vi "eDyno Fault Sequencer.vi"(0 "Automated Sequence":T5={"Run Auto Sequence"=FALSE, "Steps"=[{"Fault Injection"={"Imbalance ON"=FALSE, "Imbalance (g)"=0.5, "Misalignment ON"=FALSE, "Misalignment (g)"=0.2, "Bearing BPFO ON"=FALSE, "Bearing Impact (g)"=2.0, "Motor Ripple ON"=FALSE, "Torque Ripple (g)"=0.3, "PWM Noise ON"=FALSE, "PWM Level (g)"=0.05}, "Speed Profile"={"Run-up Enabled"=TRUE, "Constant Speed (rpm)"=3000.0, "Run-up Start (rpm)"=500.0, "Run-up End (rpm)"=4500.0, "Run-up Duration (s)"=30.0}, "Dwell (s)"=32.0}, {"Fault Injection"={"Imbalance ON"=TRUE, "Imbalance (g)"=0.5, "Misalignment ON"=FALSE, "Misalignment (g)"=0.2, "Bearing BPFO ON"=FALSE, "Bearing Impact (g)"=2.0, "Motor Ripple ON"=FALSE, "Torque Ripple (g)"=0.3, "PWM Noise ON"=FALSE, "PWM Level (g)"=0.05}, "Speed Profile"={"Run-up Enabled"=TRUE, "Constant Speed (rpm)"=3000.0, "Run-up Start (rpm)"=500.0, "Run-up End (rpm)"=4500.0, "Run-up Duration (s)"=30.0}, "Dwell (s)"=32.0}, {"Fault Injection"={"Imbalance ON"=FALSE, "Imbalance (g)"=0.5, "Misalignment ON"=TRUE, "Misalignment (g)"=0.2, "Bearing BPFO ON"=FALSE, "Bearing Impact (g)"=2.0, "Motor Ripple ON"=FALSE, "Torque Ripple (g)"=0.3, "PWM Noise ON"=FALSE, "PWM Level (g)"=0.05}, "Speed Profile"={"Run-up Enabled"=TRUE, "Constant Speed (rpm)"=3000.0, "Run-up Start (rpm)"=500.0, "Run-up End (rpm)"=4500.0, "Run-up Duration (s)"=30.0}, "Dwell (s)"=32.0}, {"Fault Injection"={"Imbalance ON"=FALSE, "Imbalance (g)"=0.5, "Misalignment ON"=FALSE, "Misalignment (g)"=0.2, "Bearing BPFO ON"=TRUE, "Bearing Impact (g)"=2.0, "Motor Ripple ON"=FALSE, "Torque Ripple (g)"=0.3, "PWM Noise ON"=FALSE, "PWM Level (g)"=0.05}, "Speed Profile"={"Run-up Enabled"=TRUE, "Constant Speed (rpm)"=3000.0, "Run-up Start (rpm)"=500.0, "Run-up End (rpm)"=4500.0, "Run-up Duration (s)"=30.0}, "Dwell (s)"=32.0}, {"Fault Injection"={"Imbalance ON"=FALSE, "Imbalance (g)"=0.5, "Misalignment ON"=FALSE, "Misalignment (g)"=0.2, "Bearing BPFO ON"=FALSE, "Bearing Impact (g)"=2.0, "Motor Ripple ON"=TRUE, "Torque Ripple (g)"=0.3, "PWM Noise ON"=FALSE, "PWM Level (g)"=0.05}, "Speed Profile"={"Run-up Enabled"=TRUE, "Constant Speed (rpm)"=3000.0, "Run-up Start (rpm)"=500.0, "Run-up End (rpm)"=4500.0, "Run-up Duration (s)"=30.0}, "Dwell (s)"=32.0}, {"Fault Injection"={"Imbalance ON"=FALSE, "Imbalance (g)"=0.5, "Misalignment ON"=FALSE, "Misalignment (g)"=0.2, "Bearing BPFO ON"=FALSE, "Bearing Impact (g)"=2.0, "Motor Ripple ON"=FALSE, "Torque Ripple (g)"=0.3, "PWM Noise ON"=TRUE, "PWM Level (g)"=0.05}, "Speed Profile"={"Run-up Enabled"=TRUE, "Constant Speed (rpm)"=3000.0, "Run-up Start (rpm)"=500.0, "Run-up End (rpm)"=4500.0, "Run-up Duration (s)"=30.0}, "Dwell (s)"=32.0}]}, 5 "Panel Fault Injection":T4={"Imbalance ON"=FALSE, "Imbalance (g)"=0.5, "Misalignment ON"=FALSE, "Misalignment (g)"=0.2, "Bearing BPFO ON"=FALSE, "Bearing Impact (g)"=2.0, "Motor Ripple ON"=FALSE, "Torque Ripple (g)"=0.3, "PWM Noise ON"=FALSE, "PWM Level (g)"=0.05}, 7 "Panel Speed Profile":T3={"Run-up Enabled"=FALSE, "Constant Speed (rpm)"=3000.0, "Run-up Start (rpm)"=500.0, "Run-up End (rpm)"=4500.0, "Run-up Duration (s)"=30.0}, 9 "Block Duration (s)":dbl=0.1, 11 "State in":T1) -> (4 "Fault Injection":T4={"Imbalance ON"=FALSE, "Imbalance (g)"=0.5, "Misalignment ON"=FALSE, "Misalignment (g)"=0.2, "Bearing BPFO ON"=FALSE, "Bearing Impact (g)"=2.0, "Motor Ripple ON"=FALSE, "Torque Ripple (g)"=0.3, "PWM Noise ON"=FALSE, "PWM Level (g)"=0.05}, 6 "Speed Profile":T3={"Run-up Enabled"=FALSE, "Constant Speed (rpm)"=3000.0, "Run-up Start (rpm)"=500.0, "Run-up End (rpm)"=4500.0, "Run-up Duration (s)"=30.0}, 8 "Restart Run-up":bool, 10 "Sequence Status":T2, 15 "State out":T1)   [LabVIEW 2026]
doc: "Fault/speed step sequencer for the eDyno NVH simulator, called once per AO block. Keep State in/out in a shift register initialised to [0,0,0,0]. Run Auto Sequence OFF: passes the panel Fault Injection and Speed Profile through (Seq State 0 = Manual). ON: applies Steps[i] and moves to the next step after Dwell (s); after the last step it falls back to the panel values (Seq State 3 = AutoDone). Seq State 2 = AutoRunning. Restart Run-up is TRUE on the block where a step starts (or the mode changes) - reset the speed-profile time to 0 there. Test Step increments on every such change."
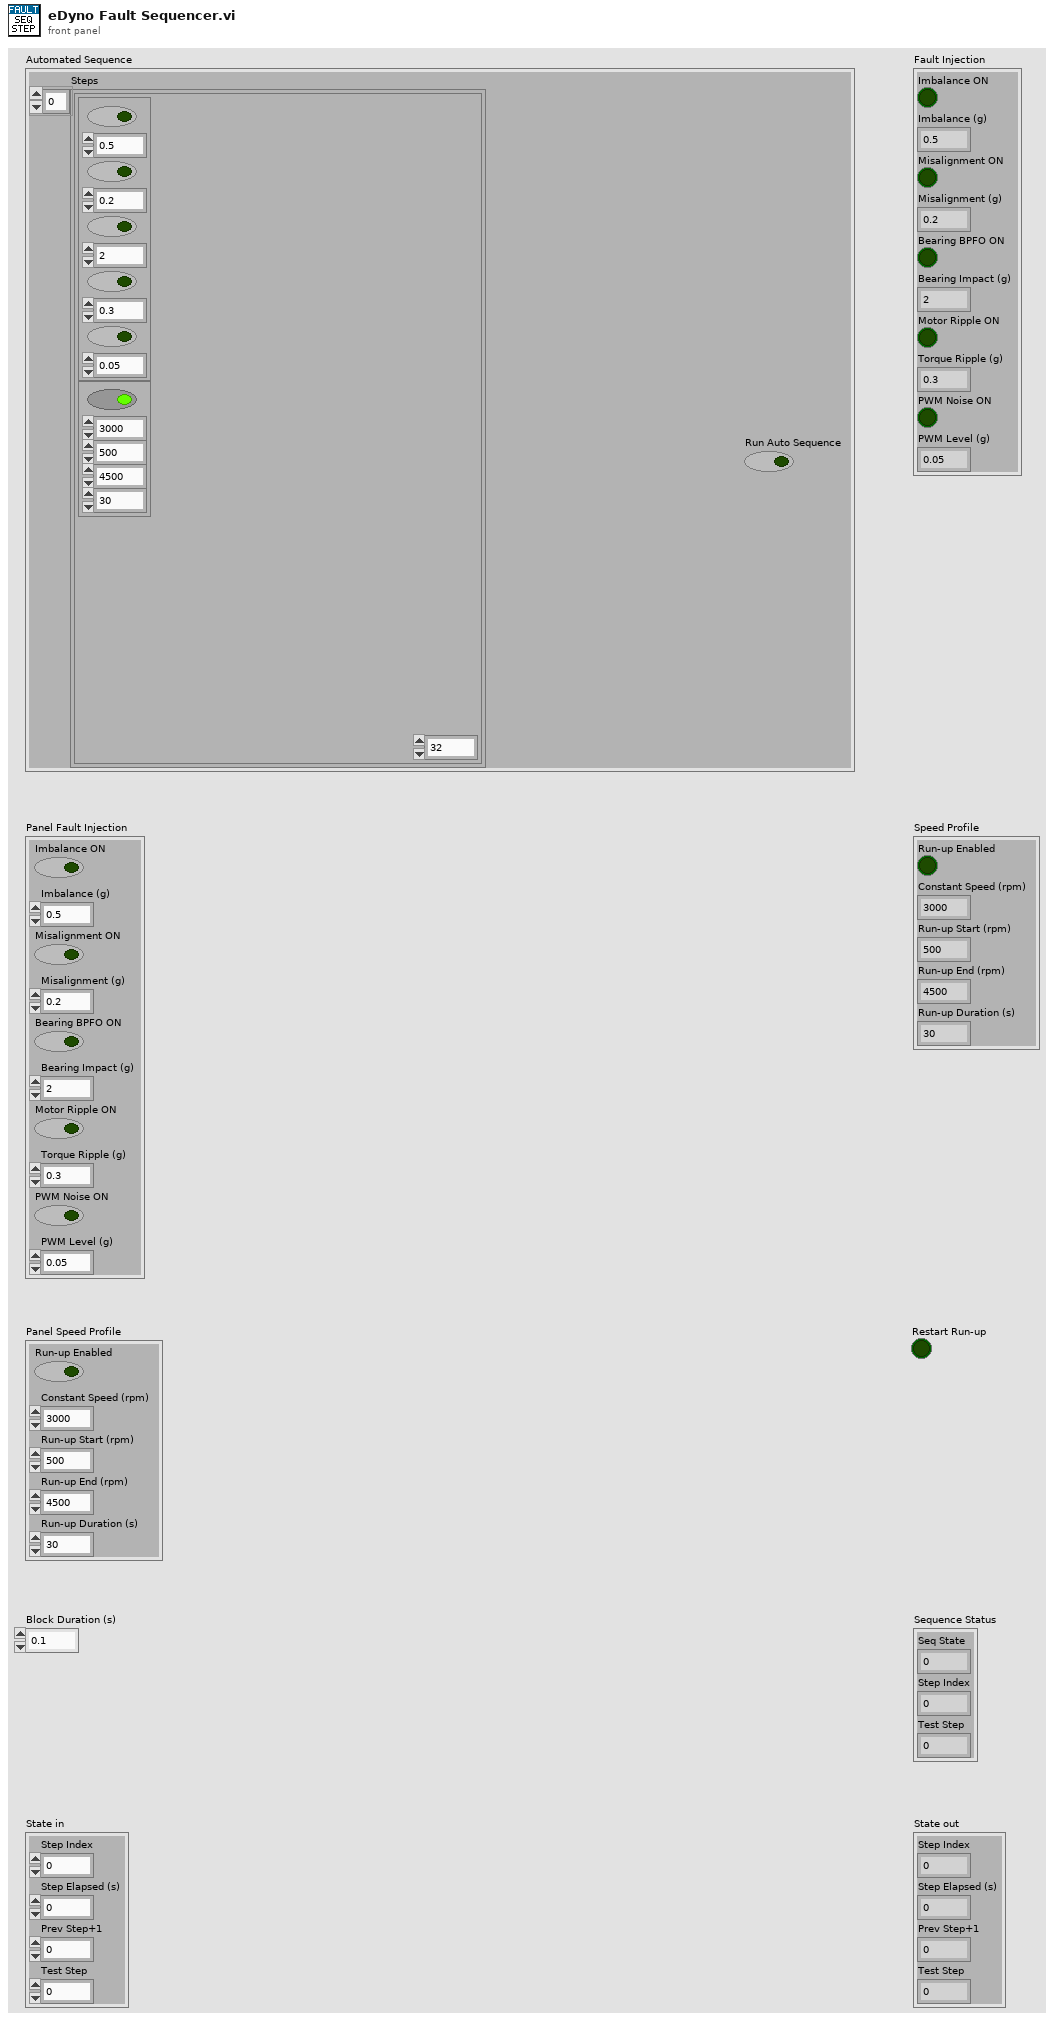
[diagram p1: front panel]
types:
  T1 = cluster{"Step Index":i32, "Step Elapsed (s)":dbl, "Prev Step+1":i32, "Test Step":dbl}
  T2 = cluster{"Seq State":dbl, "Step Index":i32, "Test Step":dbl}
  T3 = cluster{"Run-up Enabled":bool, "Constant Speed (rpm)":dbl, "Run-up Start (rpm)":dbl, "Run-up End (rpm)":dbl, "Run-up Duration (s)":dbl}
  T4 = cluster{"Imbalance ON":bool, "Imbalance (g)":dbl, "Misalignment ON":bool, "Misalignment (g)":dbl, "Bearing BPFO ON":bool, "Bearing Impact (g)":dbl, "Motor Ripple ON":bool, "Torque Ripple (g)":dbl, "PWM Noise ON":bool, "PWM Level (g)":dbl}
  T5 = cluster{"Run Auto Sequence":bool, "Steps":cluster{"Fault Injection":cluster{"Imbalance ON":bool, "Imbalance (g)":dbl, "Misalignment ON":bool, "Misalignment (g)":dbl, "Bearing BPFO ON":bool, "Bearing Impact (g)":dbl, "Motor Ripple ON":bool, "Torque Ripple (g)":dbl, "PWM Noise ON":bool, "PWM Level (g)":dbl}, "Speed Profile":cluster{"Run-up Enabled":bool, "Constant Speed (rpm)":dbl, "Run-up Start (rpm)":dbl, "Run-up End (rpm)":dbl, "Run-up Duration (s)":dbl}, "Dwell (s)":dbl}[]}
  T6 = cluster{"Fault Injection":cluster{"Imbalance ON":bool, "Imbalance (g)":dbl, "Misalignment ON":bool, "Misalignment (g)":dbl, "Bearing BPFO ON":bool, "Bearing Impact (g)":dbl, "Motor Ripple ON":bool, "Torque Ripple (g)":dbl, "PWM Noise ON":bool, "PWM Level (g)":dbl}, "Speed Profile":cluster{"Run-up Enabled":bool, "Constant Speed (rpm)":dbl, "Run-up Start (rpm)":dbl, "Run-up End (rpm)":dbl, "Run-up Duration (s)":dbl}, "Dwell (s)":dbl}[]
  T7 = cluster{"Fault Injection":cluster{"Imbalance ON":bool, "Imbalance (g)":dbl, "Misalignment ON":bool, "Misalignment (g)":dbl, "Bearing BPFO ON":bool, "Bearing Impact (g)":dbl, "Motor Ripple ON":bool, "Torque Ripple (g)":dbl, "PWM Noise ON":bool, "PWM Level (g)":dbl}, "Speed Profile":cluster{"Run-up Enabled":bool, "Constant Speed (rpm)":dbl, "Run-up Start (rpm)":dbl, "Run-up End (rpm)":dbl, "Run-up Duration (s)":dbl}, "Dwell (s)":dbl}
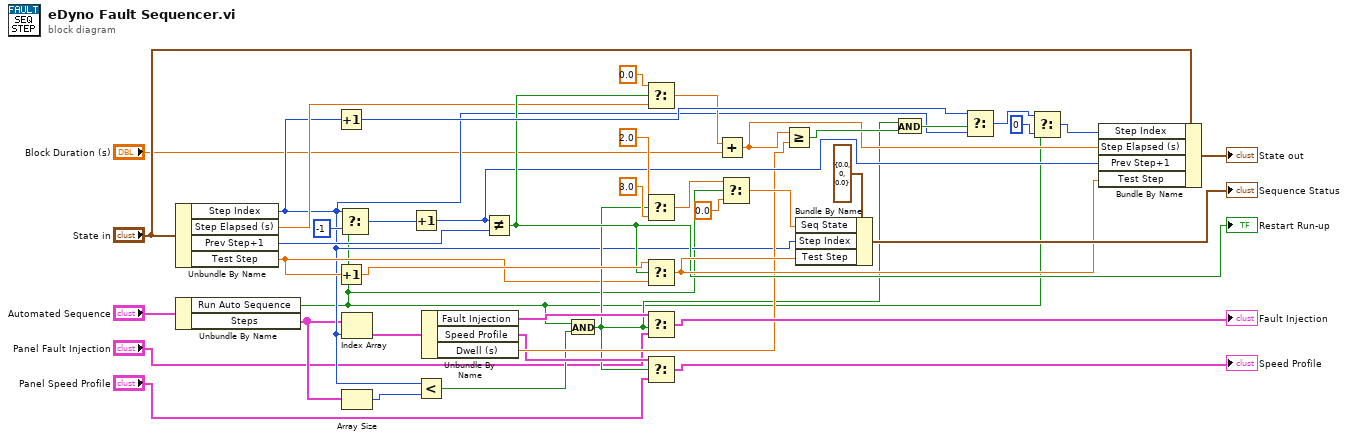
[diagram p0: block diagram]
diagram:
  n1 = Unbundle By Name("State in") -> ("Step Index"=w8:i32, "Step Elapsed (s)"=w9:dbl, "Prev Step+1"=w10:i32, "Test Step"=w11:dbl)
  n2 = Unbundle By Name("Automated Sequence") -> ("Run Auto Sequence"=w6:bool, "Steps"=w7:T6)
  n3 = Increment(x=w8) -> (x+1=w31:i32)
  n4 = Increment(x=w11) -> (x+1=w34:dbl)
  n5 = Select(t=w8, s=w6, f=-1 ("minus one")) -> (s? t:f=w23:i32)
  n6 = Index Array(array=w7, index=w8) -> (element=w15:T7)
  n7 = Array Size(array=w7) -> (size(s)=w12:i32)
  n8 = Increment(x=w23) -> (x+1=w24:i32)
  n9 = Less?(x=w8, y=w12) -> (x < y?=w13:bool)
  n10 = Unbundle By Name(w15) -> ("Fault Injection"=w16:T4, "Speed Profile"=w17:T3, "Dwell (s)"=w18:dbl)
  n11 = Not Equal?(x=w24, y=w10) -> (x != y?=w25:bool)
  "Restart Run-up" <- w25
  n12 = And(x=w6, y=w13) -> (x .and. y?=w14:bool)
  n13 = Select(t=0.0 ("zero s"), s=w25, f=w9) -> (s? t:f=w27:dbl)
  n14 = Select(t=2.0 ("AutoRunning"), s=w14, f=3.0 ("AutoDone")) -> (s? t:f=w39:dbl)
  n15 = Select(t=w34, s=w25, f=w11) -> (s? t:f=w35:dbl)
  n16 = Select(t=w16, s=w14, f="Panel Fault Injection") -> (s? t:f=→"Fault Injection":T4)
  n17 = Select(t=w17, s=w14, f="Panel Speed Profile") -> (s? t:f=→"Speed Profile":T3)
  n18 = Add(x=w27, y="Block Duration (s)") -> (x+y=w28:dbl)
  n19 = Select(t=w39, s=w6, f=0.0 ("Manual")) -> (s? t:f=w40:dbl)
  n20 = Greater Or Equal?(x=w28, y=w18) -> (x >= y?=w29:bool)
  n21 = Bundle By Name(cluster=T2 {"Seq State"=0.0, "Step Index"=0, "Test Step"=0.0} ("status"), "Seq State"=w40, "Step Index"=w8, "Test Step"=w35) -> (→"Sequence Status":T2)
  n22 = And(x=w14, y=w29) -> (x .and. y?=w30:bool)
  n23 = Select(t=w31, s=w30, f=w8) -> (s? t:f=w32:i32)
  n24 = Select(t=w32, s=w6, f=0 ("zero")) -> (s? t:f=w33:i32)
  n25 = Bundle By Name(cluster="State in", "Step Index"=w33, "Step Elapsed (s)"=w28, "Prev Step+1"=w24, "Test Step"=w35) -> (→"State out":T1)
